vi "Motor_Create Single AI.vi"(6 "Signal_Type":string="Signal_Type", 7 "section":string="Motor", 8 "error in (no error)":errorcluster, 9 "AI_Range":string="Speed_AI_Range", 10 "AI_Channel":string="Speed_AI_Channel", 11 "Path In":path) -> (0 "error out":errorcluster, 2 "AnalogInput.lvclass":refnum<class "AnalogInput.lvclass">, 3 "Path Out":path)   [LabVIEW 2021]
uses:
  AnalogInput/AnalogInput.lvclass
  Modbus_AI/Modbus_AI.lvclass
  C:/Users/lincoln.lucio/Documents/Lincoln/Documentos Pessoais/meus docs/Projetos pessoais/Projeto Sciranda/projeto_versioned/sciranda/AnalogInput/AnalogInput.lvclass
  Modbus_Master/Modbus_Master.lvclass
  Modbus_AI/Modbus_AI.lvclass/Modbus_AI.ctl
  DAQNavi_AI.lvclass/DAQNavi_AI.lvclass
  DAQNavi_AI.lvclass/DAQNavi_AI.lvclass/DAQNavi_AI.ctl
  Modbus_AI/Accessor VIs/Write Modbus_Master.lvclass.vi
  Modbus_AI/Accessor VIs/Write Register Address.vi
  Modbus_AI/Accessor VIs/Write Is Signed (I16)_.vi
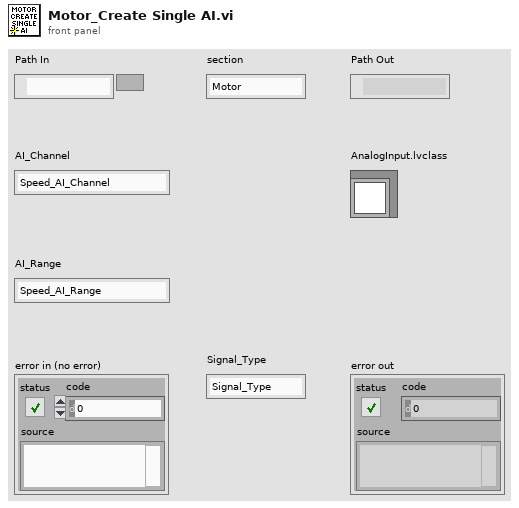
[diagram p1: front panel]
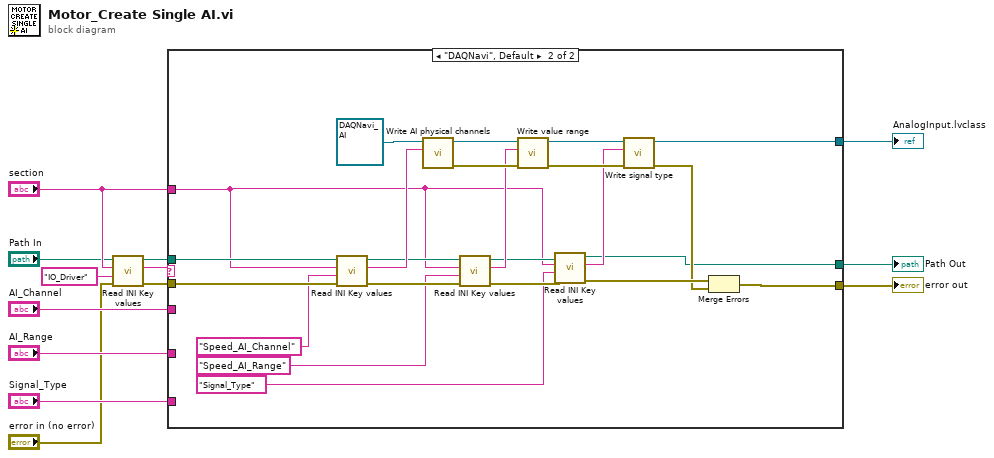
[diagram p0: block diagram]
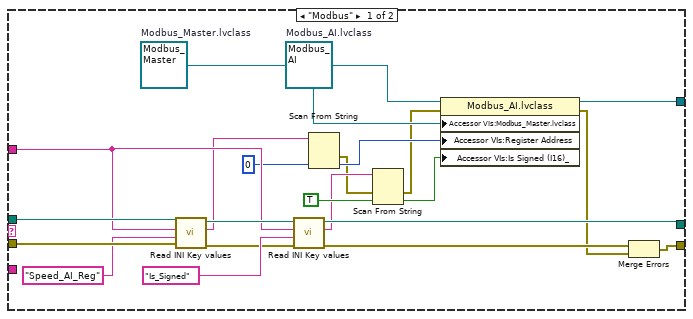
[diagram p2: hidden frame]
diagram:
  n1 = call "Read INI Key values.vi"("error in (no error)"="error in (no error)", "key"="IO_Driver", "section"="section", "Path In"="Path In") -> ("error out"=w3:errorcluster, "value"=w8:string, "Path Out"=w5:path)  [unwired: 5 in]
  n2 = case shown="\"DAQNavi\", Default" w8 {
    tunnel: w5 -> [w35 w57]
    tunnel: "AI_Channel" -> [_ _]
    tunnel: "AI_Range" -> [_ _]
    tunnel: "section" -> [w27 w46]
    tunnel: "Signal_Type" -> [_ _]
    tunnel: w3 -> [w34 w44]
    tunnel: [w15 w41] -> w10
    tunnel: [w25 w40] -> w1
    tunnel: [w29 w39] -> w9
    frame "Modbus" {
      w24 = refnum<class "Modbus_Master.lvclass"> refnum  # Modbus_Master.lvclass
      w26 = refnum<class "Modbus_AI.lvclass"> refnum  # Modbus_AI.lvclass
      n3 = call "Read INI Key values.vi"("error in (no error)"=w34, "key"="Speed_AI_Reg", "section"=w27, "Path In"=w35) -> ("error out"=w30:errorcluster, "value"=w22:string, "Path Out"=w31:path)  [unwired: 5 in]
      n4 = call "Read INI Key values.vi"("error in (no error)"=w30, "key"="Is_Signed", "section"=w27, "Path In"=w31) -> ("error out"=w28:errorcluster, "value"=w19:string, "Path Out"=w29:path)  [unwired: 5 in]
      n5 = Scan From String(input string=w22, default 1=u16 0 ("Register Address")) -> (error out=w17:errorcluster, output 1=w21:u16)  [unwired: 3 in, 2 out]
      n6 = Scan From String(input string=w19, error in=w17, default 1=TRUE ("Is Signed (I16)_")) -> (error out=w16:errorcluster, output 1=w18:bool)  [unwired: 2 in, 2 out]
      n7 = property class="Modbus_AI.lvclass"(reference=w26, error in=w16, "Accessor VIs:Modbus_Master.lvclass"=w24, "Accessor VIs:Register Address"=w21, "Accessor VIs:Is Signed (I16)_"=w18) -> (reference out=w25:refnum<class "Modbus_AI.lvclass">, error out=w14:errorcluster)
      n8 = Merge Errors(w28, w14) -> (w15:errorcluster)
    }
    frame "DAQNavi", Default {
      n9 = call "Read INI Key values.vi"("error in (no error)"=w44, "key"="Speed_AI_Channel" ("AI_Channel"), "section"=w46, "Path In"=w57) -> ("error out"=w54:errorcluster, "value"=w56:string, "Path Out"=w55:path)  [unwired: 5 in]
      n10 = call "Write AI physical channels.vi"("physical channels"=w56, "DAQNavi_AI in"=refnum<class "DAQNavi_AI.lvclass"> refnum ("DAQNavi_AI.lvclass")) -> ("error out"=w52:errorcluster, "DAQNavi_AI out"=w53:refnum<class "DAQNavi_AI.lvclass">)  [unwired: 8 in]
      n11 = call "Read INI Key values.vi"("error in (no error)"=w54, "key"="Speed_AI_Range" ("AI_Range"), "section"=w46, "Path In"=w55) -> ("error out"=w47:errorcluster, "value"=w49:string, "Path Out"=w48:path)  [unwired: 5 in]
      n12 = call "Write value range.vi"("error in (no error)"=w52, "value range"=w49, "DAQNavi_AI in"=w53) -> ("error out"=w50:errorcluster, "DAQNavi_AI out"=w51:refnum<class "DAQNavi_AI.lvclass">)  [unwired: 7 in]
      n13 = call "Read INI Key values.vi"("error in (no error)"=w47, "key"="Signal_Type" ("Signal_Type"), "section"=w46, "Path In"=w48) -> ("error out"=w43:errorcluster, "value"=w45:string, "Path Out"=w39:path)  [unwired: 5 in]
      n14 = call "Write signal type.vi"("error in (no error)"=w50, "signal type"=w45, "DAQNavi_AI in"=w51) -> ("error out"=w42:errorcluster, "DAQNavi_AI out"=w40:refnum<class "DAQNavi_AI.lvclass">)  [unwired: 7 in]
      n15 = Merge Errors(w43, w42) -> (w41:errorcluster)
    }
  }
  "error out" <- w10
  "Path Out" <- w9
  "AnalogInput.lvclass" <- w1
